vi "KYFG Camera Scan.vi"(8 "error in (no error)":errorcluster, 11 "handle":u32) -> (0 "error out":errorcluster, 1 "detectedCameras out":i32, 2 "camHandleArray":u32[](array[numeric]))   [LabVIEW 2023]
doc: "KYFG_API FGSTATUS KYFG_CameraScan(FGHANDLE handle, CAMHANDLE *camHandleArray, int *detectedCameras);"
uses:
  KYFGLib_lv.lvlib
  KYFGLib.dll
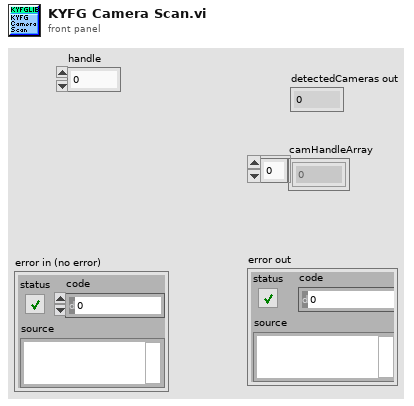
[diagram p1: front panel]
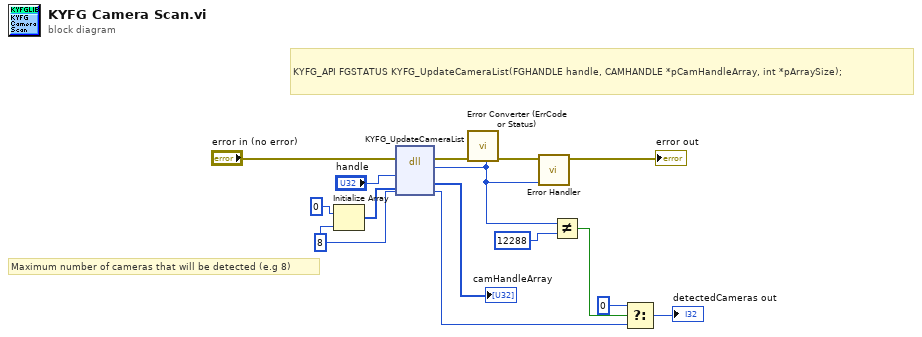
[diagram p0: block diagram]
diagram:
  w3 = 8 ("dimension size")
  # "Maximum number of cameras that will be detected (e.g 8)"
  # "KYFG_API FGSTATUS KYFG_UpdateCameraList(FGHANDLE handle, CAMHANDLE *pCamHandleArray, int *pArraySize);"
  n1 = Initialize Array(0, w3) -> (w4:i32[])
  n2 = dll-call lib="KYFGLib.dll" fn="KYFG_UpdateCameraList"(error in="error in (no error)", "handle"="handle", "camHandleArray"=w4, "detectedCameras"=w3) -> (error out=w12:errorcluster, "return type"=w1:u32, "camHandleArray"=→"camHandleArray":u32[], "detectedCameras"=w7:i32)  [unwired: 3 in, 1 out]
  n3 = call "Error Converter (ErrCode or Status).vi"("error in (no error)"=w12, "error code"=w1) -> ("error out"=w11:errorcluster)  [unwired: 9 in]
  n4 = call "Error Handler.vi"("Return Code"=w1, "Error In"=w11) -> ("Error Out"=→"error out":errorcluster)  [unwired: 9 in]
  n5 = Not Equal?(x=w1, y=u32 12288) -> (x != y?=w9:bool)
  n6 = Select(t=0, s=w9, f=w7) -> (s? t:f=→"detectedCameras out":i32)
